vi "ISO 8601 UTC to Timestamp.vi"(8 "error in (no error)":errorcluster, 11 "ISO 8601 UTC":string) -> (0 "error out":errorcluster, 3 "Timestamp":timestamp)   [LabVIEW 2020, in "Time Management.lvlib"]
doc: "Parses an ISO 8601 UTC string of the form YYYY-MM-DDTHH:MM:SS.mmmZ (as written by Timestamp to ISO 8601 UTC.vi) into a timestamp. An empty string returns timestamp 0 with no error - the storage layer uses that for the End Time of a running entry. Any other string that does not match the pattern returns timestamp 0 and error 5001. Parsing uses fixed character positions and integer conversion only, so it does not depend on the Windows decimal-separator setting.\n\nGenerated by: Claude"
uses:
  Time Management.lvlib
  <vilib>/Utility/error.llb/Trim Whitespace One-Sided.vi
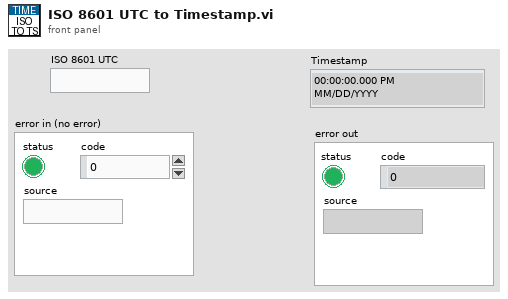
[diagram p1: front panel]
types:
  T1 = typedef "LVDateTimeRec.ctl" = cluster{"fractional second":dbl, "second":i32, "minute":i32, "hour":i32, "day of month":i32, "month":i32, "year":i32, "day of week":i32, "day of year":i32, "DST":i32}
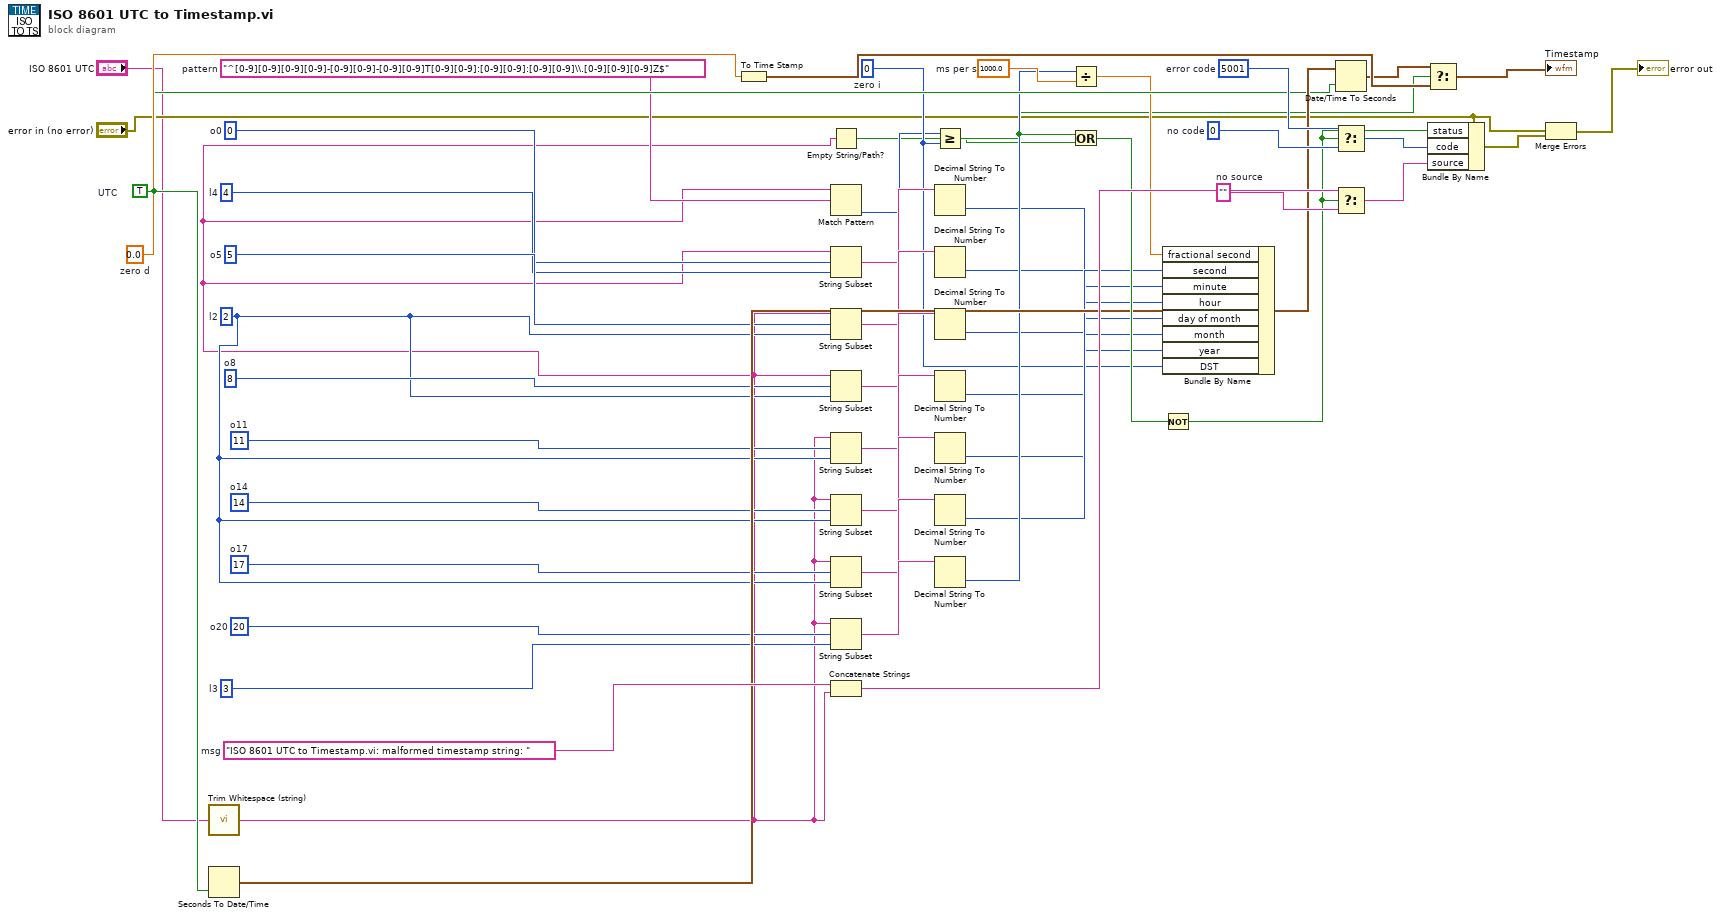
[diagram p0: block diagram]
diagram:
  w48 = ""  # no source
  w47 = 0  # no code
  w45 = "ISO 8601 UTC to Timestamp.vi: malformed timestamp string: "  # msg
  w44 = 5001  # error code
  w39 = 0.0  # zero d
  w35 = TRUE  # UTC
  w33 = 1000.0  # ms per s
  w18 = 3  # l3
  w17 = 20  # o20
  w16 = 17  # o17
  w15 = 14  # o14
  w14 = 11  # o11
  w13 = 8  # o8
  w12 = 2  # l2
  w11 = 5  # o5
  w10 = 4  # l4
  w9 = 0  # o0
  w7 = 0  # zero i
  w5 = "^[0-9][0-9][0-9][0-9]-[0-9][0-9]-[0-9][0-9]T[0-9][0-9]:[0-9][0-9]:[0-9][0-9]\\.[0-9][0-9][0-9]Z$"  # pattern
  n1 = call <vilib>:"Trim Whitespace (string).vi"("string"="ISO 8601 UTC") -> ("trimmed string"=w3:string)  [unwired: 1 in]
  n2 = Seconds To Date/Time(to UTC (F)=w35) -> (date time rec=w36:T1)  [unwired: 1 in]
  n3 = To Time Stamp(1:w39) -> (0:w40:timestamp)
  n4 = Empty String/Path?(string/path=w3) -> (empty?=w4:bool)
  n5 = Match Pattern(string=w3, regular expression=w5) -> (offset past match=w6:i32)  [unwired: 1 in, 3 out]
  n6 = String Subset(string=w3, offset (0)=w9, length (rest)=w10) -> (substring=w19:string)
  n7 = String Subset(string=w3, offset (0)=w11, length (rest)=w12) -> (substring=w20:string)
  n8 = String Subset(string=w3, offset (0)=w13, length (rest)=w12) -> (substring=w21:string)
  n9 = String Subset(string=w3, offset (0)=w14, length (rest)=w12) -> (substring=w22:string)
  n10 = String Subset(string=w3, offset (0)=w15, length (rest)=w12) -> (substring=w23:string)
  n11 = String Subset(string=w3, offset (0)=w16, length (rest)=w12) -> (substring=w24:string)
  n12 = String Subset(string=w3, offset (0)=w17, length (rest)=w18) -> (substring=w25:string)
  n13 = Concatenate Strings(w45, w3) -> (w46:string)
  n14 = Greater Or Equal?(x=w6, y=w7) -> (x >= y?=w8:bool)
  n15 = Decimal String To Number(string=w19) -> (number=w26:i32)  [unwired: 2 in, 1 out]
  n16 = Decimal String To Number(string=w20) -> (number=w27:i32)  [unwired: 2 in, 1 out]
  n17 = Decimal String To Number(string=w21) -> (number=w28:i32)  [unwired: 2 in, 1 out]
  n18 = Decimal String To Number(string=w22) -> (number=w29:i32)  [unwired: 2 in, 1 out]
  n19 = Decimal String To Number(string=w23) -> (number=w30:i32)  [unwired: 2 in, 1 out]
  n20 = Decimal String To Number(string=w24) -> (number=w31:i32)  [unwired: 2 in, 1 out]
  n21 = Decimal String To Number(string=w25) -> (number=w32:i32)  [unwired: 2 in, 1 out]
  n22 = Divide(x=w32, y=w33) -> (x/y=w34:dbl)
  n23 = Or(x=w8, y=w4) -> (x .or. y?=w42:bool)
  n24 = Bundle By Name(cluster=w36, "fractional second"=w34, "second"=w31, "minute"=w30, "hour"=w29, "day of month"=w28, "month"=w27, "year"=w26, "DST"=w7) -> (w37:T1)
  n25 = Not(x=w42) -> (.not. x?=w43:bool)
  n26 = Date/Time To Seconds(1:w35, 2:w37) -> (0:w38:timestamp)
  n27 = Select(t=w44, s=w43, f=w47) -> (s? t:f=w49:i32)
  n28 = Select(t=w46, s=w43, f=w48) -> (s? t:f=w50:string)
  n29 = Select(t=w38, s=w8, f=w40) -> (s? t:f=→"Timestamp":timestamp)
  n30 = Bundle By Name(cluster="error in (no error)", "status"=w43, "code"=w49, "source"=w50) -> (w51:errorcluster)
  n31 = Merge Errors("error in (no error)", w51) -> (→"error out":errorcluster)
